vi "Clear Cache.vi"(8 "error in (no error)":errorcluster, 11 ".NET Refnum in":refnum<k24>) -> (0 "error out":errorcluster)   [LabVIEW 2020]
doc: "Clear cache of webview2."
uses:
  C:/Program Files (x86)/National Instruments/LabVIEW 2020/vi.lib/sklein/WebView2/Libs/Microsoft.Web.WebView2.WinForms.dll
  Program Files (x86)/National Instruments/LabVIEW 2020/vi.lib/sklein/WebView2/Libs/Microsoft.Web.WebView2.WinForms.dll
  C:/Program Files (x86)/National Instruments/LabVIEW 2020/vi.lib/sklein/WebView2/Libs/Microsoft.Web.WebView2.Core.dll
  Program Files (x86)/National Instruments/LabVIEW 2020/vi.lib/sklein/WebView2/Libs/Microsoft.Web.WebView2.Core.dll
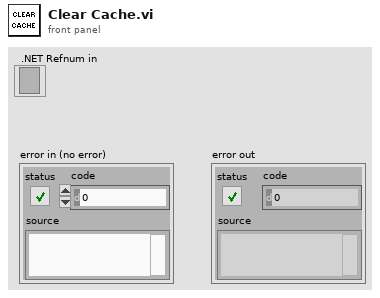
[diagram p1: front panel]
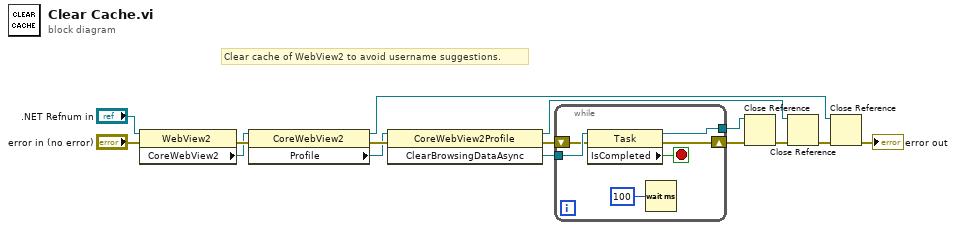
[diagram p0: block diagram]
diagram:
  # "Clear cache of WebView2 to avoid username suggestions."
  n1 = property on="Property Node" class="WebView2"(reference=".NET Refnum in", error in="error in (no error)") -> (error out=w3:errorcluster, "CoreWebView2"=w1:refnum<k24>)  [unwired: 1 out]
  n2 = property on="Property Node" class="CoreWebView2"(reference=w1, error in=w3) -> (reference out=w7:refnum<k24>, error out=w4:errorcluster, "Profile"=w2:refnum<k24>)
  n3 = invoke on="Invoke Node" class="CoreWebView2Profile" method="ClearBrowsingDataAsync"(reference=w2, error in=w4) -> (reference out=w5:refnum<k24>, error out=w12:errorcluster, "ClearBrowsingDataAsync"=w10:refnum<k24>)  [unwired: 1 in]
  n4 = while {
    tunnel: w10 -> [w21]
    tunnel: [w18] -> w11
    shift-right: [w16] -> w13
    shift-left: w12 -> [w17]
    stop <- w20 stop-if-true
    n5 = property on="Property Node" class="Task"(reference=w21, error in=w17) -> (reference out=w18:refnum<k24>, error out=w16:errorcluster, "IsCompleted"=w20:bool)
    n6 = Wait (ms)(milliseconds to wait=u32 100) -> ()  [unwired: 1 out]
  }
  n7 = Close Reference(reference=w11, error in (no error)=w13) -> (error out=w6:errorcluster)
  n8 = Close Reference(reference=w5, error in (no error)=w6) -> (error out=w8:errorcluster)
  n9 = Close Reference(reference=w7, error in (no error)=w8) -> (error out=→"error out":errorcluster)
